vi "Log Error.vi"(8 "error in":errorcluster) -> (0 "error out":errorcluster, 3 "log file path":path)   [LabVIEW 2024]
doc: "Appends one line per error to Error Log.txt in the LVTimeTracker data folder (%LOCALAPPDATA%\\LVTimeTracker), beside Projects.ini.\nLine format: timestamp TAB error code TAB error source. Line breaks in the source are replaced with spaces so each error stays on one line.\nNothing is written when error in carries no error. error out reports only a failure to write the log; the incoming error is consumed.\n\n10/2026 Erich Schlieper"
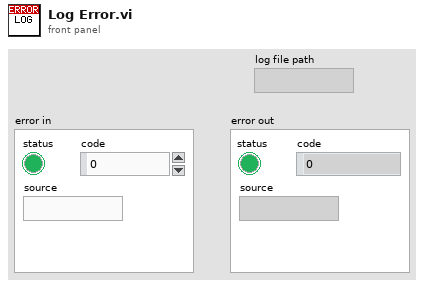
[diagram p1: front panel]
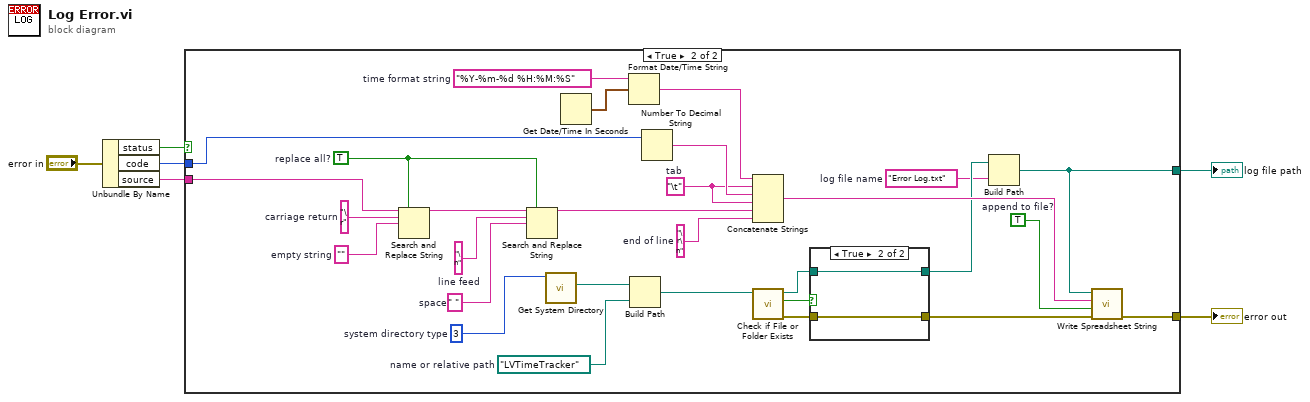
[diagram p0: block diagram]
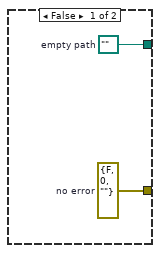
[diagram p2: hidden frame]
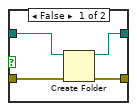
[diagram p3: hidden frame]
diagram:
  n1 = Unbundle By Name("error in") -> ("status"=w4:bool, "code"=w5:i32, "source"=w6:string)
  n2 = case shown="True" w4 {
    tunnel: w5 -> [_ w9]
    tunnel: w6 -> [_ w10]
    tunnel: [w8 w12] -> w3
    tunnel: [w7 w11] -> w2
    frame False {
      w8 = path ""  # empty path
      w7 = errorcluster {"status"=FALSE, "code"=0, "source"=""}  # no error
    }
    frame True {
      w24 = TRUE  # append to file?
      w23 = TRUE  # replace all?
      w22 = ""  # empty string
      w21 = " "  # space
      w20 = "\r"  # carriage return
      w19 = "\n"  # line feed
      w18 = "\r\n"  # end of line
      w17 = "\t"  # tab
      w16 = "%Y-%m-%d %H:%M:%S"  # time format string
      w15 = "Error Log.txt"  # log file name
      w14 = path "LVTimeTracker"  # name or relative path
      w13 = 3  # system directory type
      n3 = Search and Replace String(replace all?=w23, input string=w10, search string=w20, replace string=w22) -> (result string=w35:string)  [unwired: 4 in, 3 out]
      n4 = Search and Replace String(replace all?=w23, input string=w35, search string=w19, replace string=w21) -> (result string=w36:string)  [unwired: 4 in, 3 out]
      n5 = call <vilib>:"Get System Directory.vi"("system directory type"=w13) -> ("system directory"=w25:path)  [unwired: 10 in]
      n6 = Get Date/Time In Seconds() -> (seconds since 1Jan1904=w32:timestamp)
      n7 = Format Date/Time String(time format string (%c)=w16, seconds (now)=w32) -> (date/time string=w33:string)  [unwired: 1 out]
      n8 = Build Path(base path=w25, name or relative path=w14) -> (appended path=w26:path)
      n9 = Number To Decimal String(number=w9) -> (decimal integer string=w34:string)  [unwired: 1 in]
      n10 = Concatenate Strings(w33, w17, w34, w17, w36, w18) -> (w37:string)
      n11 = call <vilib>:"Check if File or Folder Exists.vi"("path"=w26) -> ("error out"=w27:errorcluster, "file or folder exists?"=w28:bool, "dup path"=w29:path)  [unwired: 8 in]
      n12 = case shown="True" w28 {
        tunnel: w29 -> [w38 w42]
        tunnel: w27 -> [w39 w43]
        tunnel: [w40 w43] -> w30
        tunnel: [w41 w42] -> w31
        frame False {
          n13 = Create Folder(path (use dialog)=w38, error in=w39) -> (created path=w41:path, error out=w40:errorcluster)  [unwired: 1 in, 1 out]
        }
        frame True {
        }
      }
      n14 = Build Path(base path=w31, name or relative path=w15) -> (appended path=w12:path)
      n15 = call <vilib>:"Write Spreadsheet String.vi"("error in"=w30, "append to file? (new file:F)"=w24, "spreadsheet string"=w37, "file path (dialog if empty)"=w12) -> ("error out"=w11:errorcluster)  [unwired: 6 in, 1 out]
    }
  }
  "error out" <- w2
  "log file path" <- w3
